vi "Run.vi"() -> ()   [LabVIEW 2016, in "DronaTest.lvlib"]
uses:
  DronaTest.lvlib
panel:
  out "error out":errorcluster
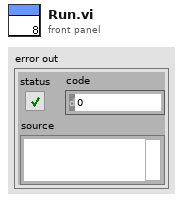
[diagram p1: front panel]
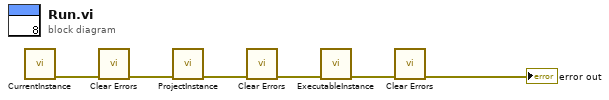
[diagram p0: block diagram]
diagram:
  n1 = call "CurrentInstance.vi"() -> ("error out"=w6:errorcluster)  [unwired: 15 in]
  n2 = call <vilib>:"Clear Errors.vi"("error in (no error)"=w6) -> ("error out"=w3:errorcluster)  [unwired: 5 in, 1 out]
  n3 = call "ProjectInstance.vi"("error in (no error)"=w3) -> ("error out"=w5:errorcluster)  [unwired: 14 in]
  n4 = call <vilib>:"Clear Errors.vi"("error in (no error)"=w5) -> ("error out"=w2:errorcluster)  [unwired: 5 in, 1 out]
  n5 = call "ExecutableInstance.vi"("error in (no error)"=w2) -> ("error out"=w4:errorcluster)  [unwired: 10 in]
  n6 = call <vilib>:"Clear Errors.vi"("error in (no error)"=w4) -> ("error out"=→"error out":errorcluster)  [unwired: 5 in, 1 out]
